vi "Clear Processes.vi"(8 "error in (no error)":errorcluster, 11 "Application In":refnum<class "Application.lvclass">) -> (0 "error out":errorcluster, 3 "Application Out":refnum<class "Application.lvclass">)   [LabVIEW 2020, in "Application.lvclass"]
uses:
  Application.lvclass
  Application.lvclass/Application.ctl
  Process/Process.lvclass
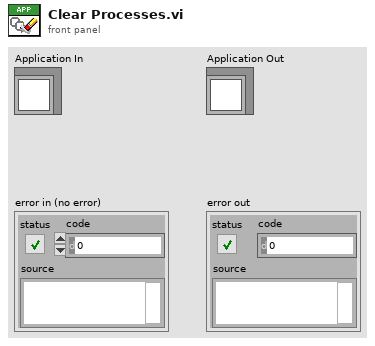
[diagram p1: front panel]
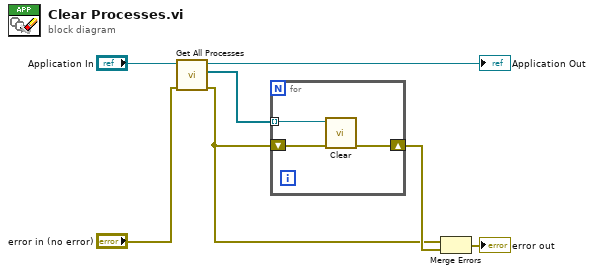
[diagram p0: block diagram]
diagram:
  n1 = call "Get All Processes.vi"("error in (no error)"="error in (no error)", "Application In"="Application In") -> ("error out"=w2:errorcluster, "App Processes"=w4:refnum<class "Process.lvclass">[], "Application Out"=→"Application Out":refnum<class "Application.lvclass">)  [unwired: 7 in]
  n2 = for {
    shift-right: [w10] -> w6
    shift-left: w2 -> [w9]
    tunnel: w4 -> [w8] mode=indexing
    n3 = call-dynamic "Clear.vi"("error in (no error)"=w9, "Process In"=w8) -> ("error out"=w10:errorcluster)  [unwired: 9 in]
  }
  n4 = Merge Errors(w2, w6) -> (→"error out":errorcluster)
